vi "DAC Configure.vi"(8 "error in":errorcluster, 11 "DAC Heater Box Temperatures in":refnum<class "DAC Heater Box Temperatures.lvclass">) -> (0 "error out":errorcluster, 3 "DAC Heater Box Temperatures out":refnum<class "DAC Heater Box Temperatures.lvclass">)   [LabVIEW 2019, in "DAC.lvlib" / "DAC Heater Box Temperatures.lvclass"]
uses:
  DAC Heater Box Temperatures.lvclass
  DAC.lvclass
  <vilib>/DAQmx/create/channels.llb/DAQmx Create Channel (AI-Temperature-RTD).vi
  <resource>/objmgr/daqmx.rc
  C:/Users/krio/Documents/LV_Projects/test-stand/App/DAC/DAC.lvclass
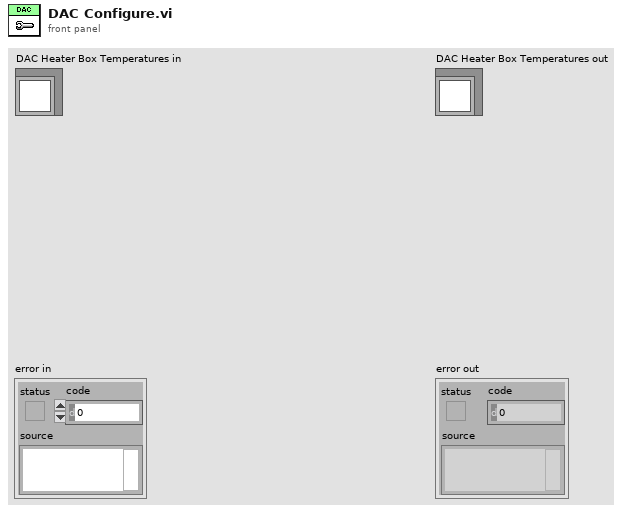
[diagram p1: front panel]
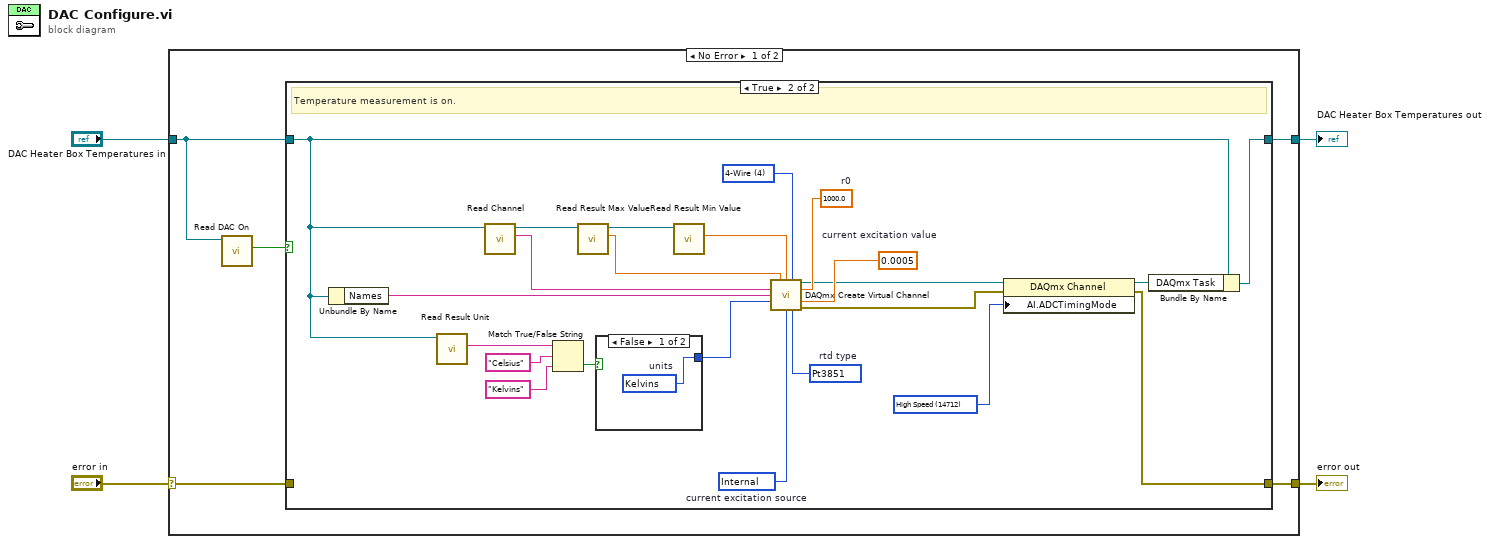
[diagram p0: block diagram]
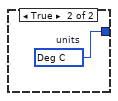
[diagram p3: hidden frame]
diagram:
  n1 = case shown="No Error" "error in" {
    selector: "error in" -> [w6 w38]
    tunnel: [w5 w38] -> w4
    tunnel: [w7 w37] -> w3
    tunnel: "DAC Heater Box Temperatures in" -> [w9 w37]
    frame No Error {
      n2 = call "Read DAC On.vi"("DAC in"=w9) -> ("DAC On"=w8:bool)  [unwired: 8 in, 2 out]
      n3 = case shown="True" w8 {
        tunnel: w9 -> [w11 w19]
        tunnel: [w11 w25] -> w7
        tunnel: w6 -> [w10 _]
        tunnel: [w10 w12] -> w5
        frame False {
          # "Temperature measurement is off."
        }
        frame True {
          w21 = 14712 items=["Automatic"=16097, "High Resolution"=10195, "High Speed"=14712, "Best 50 Hz Rejection"=14713, "Best 60 Hz Rejection"=14714, "Custom"=10137] ("AI.ADCTimingMode")
          w32 = 0.0005  # current excitation value
          w31 = 10200 items=["Internal"=10200, "External"=10167, "None"=10230]  # current excitation source
          w33 = 1000.0  # r0
          w34 = 4 items=["2-Wire"=2, "3-Wire"=3, "4-Wire"=4] ("resistance configuration")
          w30 = 10071 items=["Pt3750"=12481, "Pt3851"=10071, "Pt3911"=12482, "Pt3916"=10069, "Pt3920"=10053, "Pt3928"=12483, "Custom"=10137]  # rtd type
          # "Temperature measurement is on."
          n4 = Unbundle By Name(w19) -> ("Names"=w24:string)
          n5 = call "Read Result Unit.vi"("DAC in"=w19) -> ("Unit"=w20:string)  [unwired: 8 in, 2 out]
          n6 = call "Read Channel.vi"("DAC in"=w19) -> ("Channel"=w18:string, "DAC out"=w17:refnum<class "DAC Heater Box Temperatures.lvclass">)  [unwired: 8 in, 1 out]
          n7 = Match True/False String(2:"Kelvins" ("false string"), 3:"Celsius" ("true string"), 4:w20) -> (0:w27:bool)  [unwired: 1 out]
          n8 = call "Read Result Max Value.vi"("DAC in"=w17) -> ("Max Value"=w14:dbl, "DAC out"=w16:refnum<class "DAC Heater Box Temperatures.lvclass">)  [unwired: 8 in, 1 out]
          n9 = case shown="False" w27 {
            tunnel: [w35 w36] -> w26
            frame False {
              w35 = 10325 items=["Deg C"=10143, "Deg F"=10144, "Kelvins"=10325, "Deg R"=10145, "From Custom Scale"=10065]  # units
            }
            frame True {
              w36 = 10143 items=["Deg C"=10143, "Deg F"=10144, "Kelvins"=10325, "Deg R"=10145, "From Custom Scale"=10065]  # units
            }
          }
          n10 = call "Read Result Min Value.vi"("DAC in"=w16) -> ("Min Value"=w15:dbl)  [unwired: 8 in, 2 out]
          n11 = call-poly <vilib>:"DAQmx Create Virtual Channel.vi"("maximum value"=w14, "minimum value"=w15, "resistance configuration"=w34, "physical channels"=w18, "r0"=w33, "name to assign"=w24, "units"=w26, "current excitation value"=w32, "current excitation source"=w31, "rtd type"=w30) -> ("task out"=w23:refnum<k21>, "error out"=w13:errorcluster)  [unwired: 4 in]
          n12 = property class="DAQmx Channel"(reference=w23, error in=w13, "AI.ADCTimingMode"=w21) -> (reference out=w22:refnum<k21>, error out=w12:errorcluster)
          n13 = Bundle By Name(cluster=w19, "DAQmx Task"=w22) -> (w25:refnum<class "DAC Heater Box Temperatures.lvclass">)
        }
      }
    }
    frame Error {
    }
  }
  "error out" <- w4
  "DAC Heater Box Temperatures out" <- w3
